vi "CSE Callback - Dialog Debugger.vi"(6 "Custom data":string, 7 "VC Handle":T2=-1, 8 "error in":errorcluster, 9 "Call Reason":T1=1 items=["Exec Start", "Action completed", "pause to breath", "reserved 1", "reserved 2", "custom"], 10 "Stm Index":i32, 11 "CSE RefNum":T3) -> (0 "error out":errorcluster, 1 "Run Mode":T4 items=["Execute", "Abort", "Run", "Step", "Step Over", "Step Out", "Run (LM)", "Step (LM)", "Step Over (LM)", "Step Out (LM)", "unsupported"], 2 "Stm Index out":i32, 3 "dup CSE RefNum":T3, 4 "Breakpoints":i32[](array[numeric]), 5 "VC Handle out":T2=-1)   [LabVIEW 2021]
doc: "::: CalcExpress Toolkit :::\nCopyright (c) 2000-2026 Konstantin Shifershteyn. All rights reserved."
uses:
  vi.lib/addons/CalcExpress/cse.llb/CSE Instance RefNum.ctl
  vi.lib/addons/CalcExpress/cetypes.llb/VarMan Variable Context Handle.ctl
  vi.lib/addons/CalcExpress/cse.llb/CSE Type - Run Mode.ctl
  vi.lib/addons/CalcExpress/cse.llb/CSE Type - Callback Call Reason.ctl
  <vilib>/Utility/miscctls.llb/LVRowAndColumnTypeDef.ctl
panel:
  in  "Quick exit":bool
  in  "Exit":bool caption="EXIT"
  in  "Breakpoint":bool caption="Set Breakpoint"
  in  "Stop":bool caption="Stop Debugging"
  in  "Pause":bool
  in  "Stepping mode":bool=TRUE
  in  "Restart":bool caption="Restart Script"
  in  "GoToCursor":bool caption="Go to Cursor"
  in  "StepOut":bool caption="Step Out"
  in  "StepOver":bool caption="Step Over"
  in  "Step":bool caption="Single Step"
  in  "Run":bool caption="Run Script"
  in  "Script List":i32(listbox) caption="Script"
  out "msg":string caption="Status message"
  in  "Var List":i32(listbox) caption="Variable List (inspect variables by double-click)"
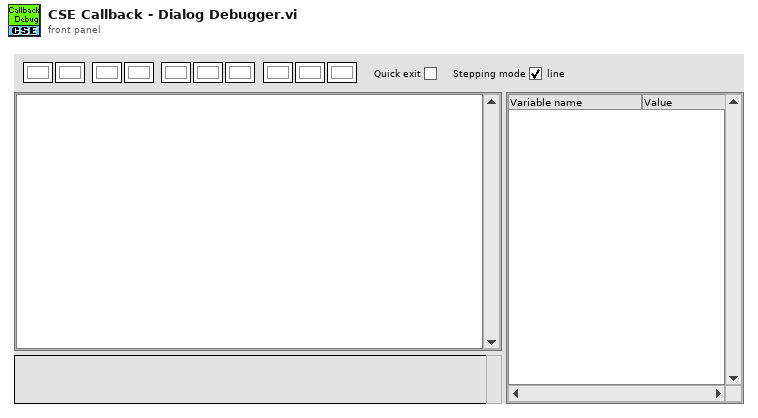
[diagram p1: front panel]
types:
  T1 = typedef "CSE Type - Callback Call Reason.ctl" = u32
  T2 = typedef "VarMan Variable Context Handle.ctl" = i32
  T3 = typedef "CSE Instance RefNum.ctl" = refnum<k1>
  T4 = typedef "CSE Type - Run Mode.ctl" = u32
  T5 = typedef "LVRowAndColumnTypeDef.ctl" = cluster{"Row":i32, "Column":i32}
  T6 = enum32{"nop", "save info", "restore info", "remove info"}
  T7 = cluster{"Selection Start":u32, "Selection End":u32}
  T8 = cluster{"level":i32, "Caller CSE RefNum":T3, "Callee CSE RefNum":T3}
  T9 = typedef "CalcExpress Instance RefNum.ctl" = refnum<k1>
  T10 = cluster{"CE InstanceRef":T9, "post action":enum32{"jump", "jump if true", "jump if false", "stop"}, "jump index":i32, "stmType":i32, "nesting level":i32, "stmOffset":i32, "stmLength":i32, "stmLine ":i32, "expOffset":i32, "expLength":i32, "expLine":i32, "parent index":i32}
  T11 = typedef "LVRowAndColumnUnsignedTypeDef.ctl" = cluster{"Row":u32, "Column":u32}
  T12 = typedef "VarMan Variable Info Cluster.ctl" = cluster{"name":string, "alias":string, "type":u32, "history":bool}
  T13 = enum8{"Enabled", "Disabled", "Disabled and Grayed Out"}
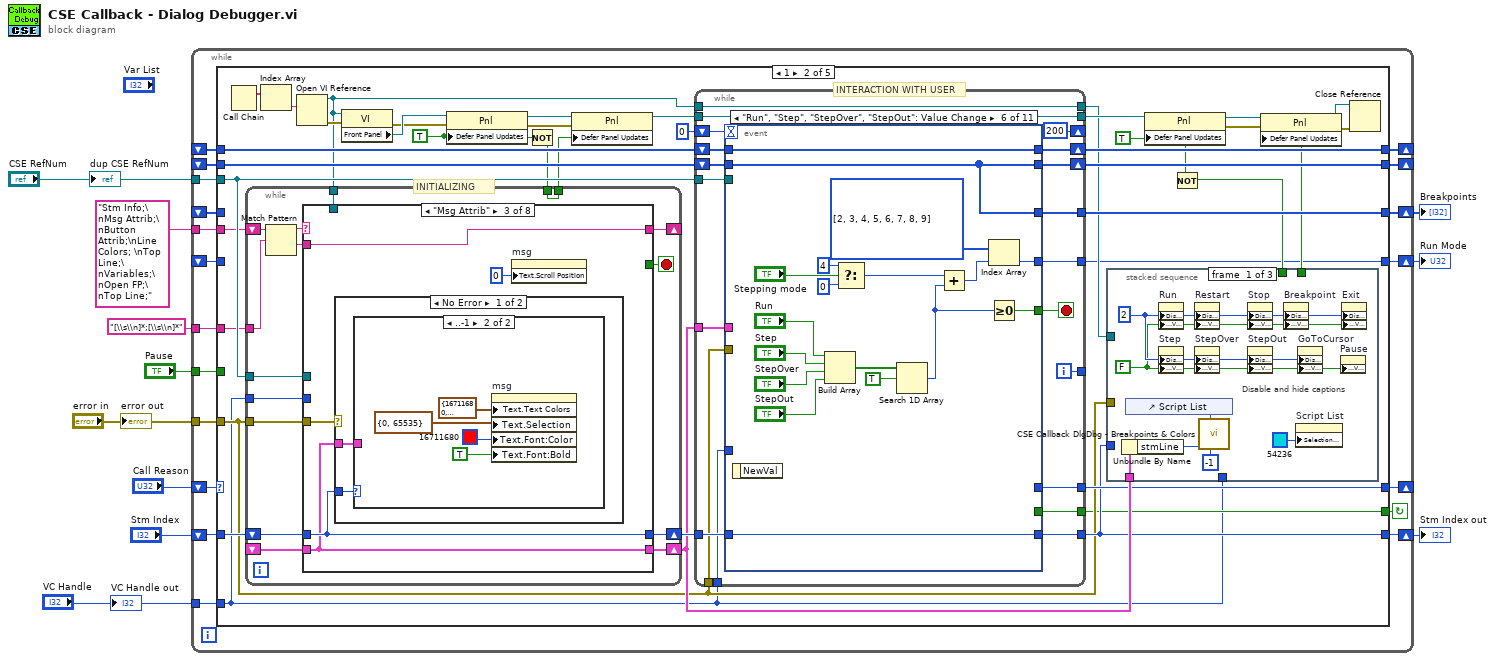
[diagram p0: block diagram]
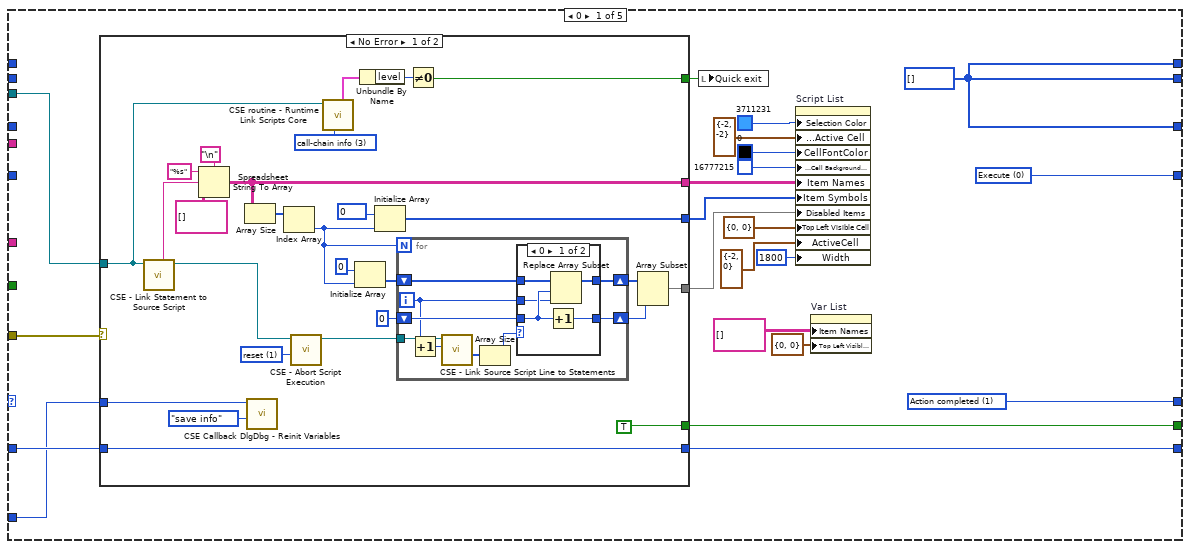
[diagram p2: hidden frame]
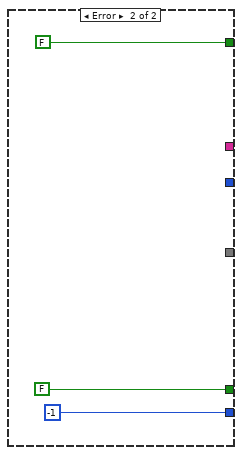
[diagram p4: hidden frame]
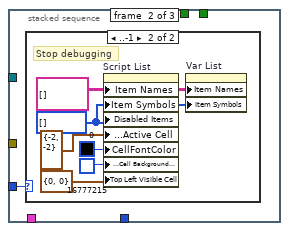
[diagram p5: hidden frame]
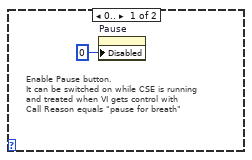
[diagram p6: hidden frame]
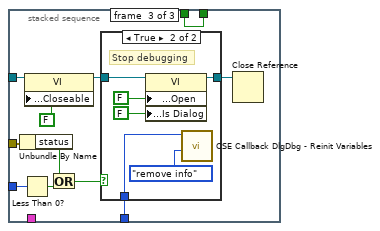
[diagram p7: hidden frame]
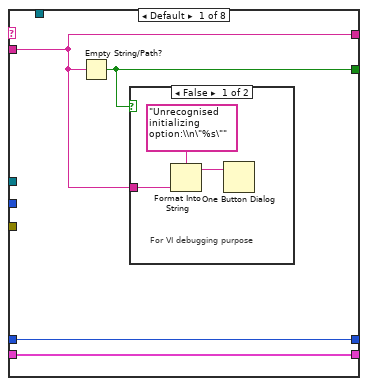
[diagram p9: hidden frame]
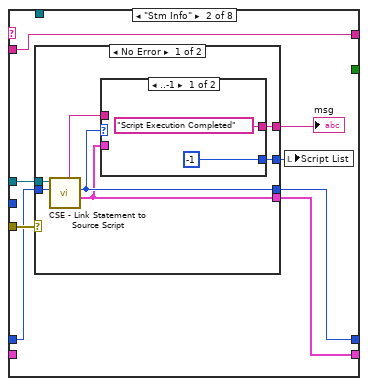
[diagram p11: hidden frame]
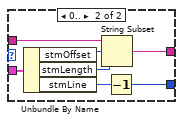
[diagram p12: hidden frame]
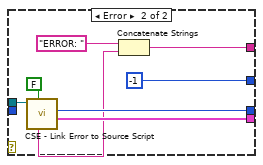
[diagram p13: hidden frame]
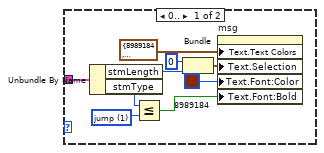
[diagram p14: hidden frame]
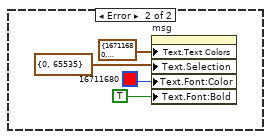
[diagram p15: hidden frame]
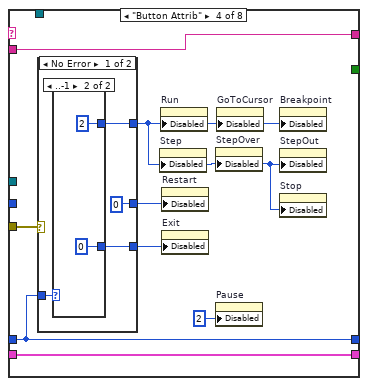
[diagram p16: hidden frame]
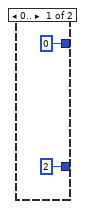
[diagram p17: hidden frame]
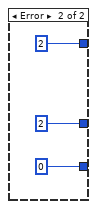
[diagram p18: hidden frame]
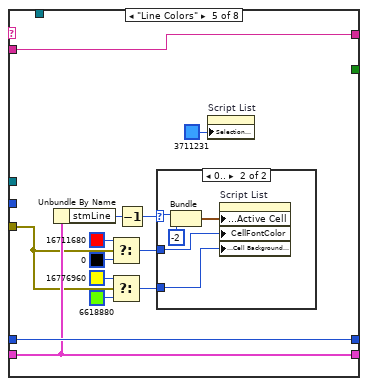
[diagram p19: hidden frame]
diagram:
  n1 = while {
    shift-right: [w29] -> _
    shift-left: "Call Reason" -> [w30]
    tunnel: "error in" -> [w27]
    tunnel: "CSE RefNum" -> [w26]
    shift-right: [w25] -> _
    shift-left: _ -> [w24]
    tunnel: "[\\s\\n]*;[\\s\\n]*" ("regular expression") -> [w23]
    tunnel: "Stm Info;\nMsg Attrib;\nButton Attrib;\nLine Colors; \nTop Line;\nVariables;\nOpen FP;\nTop Line;" -> [w22]
    shift-right: [w20] -> w5
    shift-left: "Stm Index" -> [w21]
    tunnel: "VC Handle" -> [w19]
    shift-right: [w18] -> _
    shift-left: _ -> [w17]
    tunnel: "Pause" -> [w16]
    shift-right: [w15] -> w2
    shift-left: _ -> [w13]
    shift-right: [w14] -> w1
    shift-left: _ -> [w12]
    stop <- w28 continue-if-true
    n2 = case shown="1" w30 {
      tunnel: [w36 w126 w549 _ _] -> w29
      tunnel: [w49 w103 w552 _ _] -> w28
      tunnel: [w37 w136 w550 w557 w564] -> w14
      tunnel: [w35 w102 w551 w556 w563] -> w15
      tunnel: w27 -> [w51 w104 _ _ _]
      tunnel: w26 -> [w52 w133 _ _ _]
      tunnel: [w37 w135 w555 w560 w567] -> w25
      tunnel: w24 -> [_ w134 w555 w560 w567]
      tunnel: w23 -> [_ w132 _ _ _]
      tunnel: w22 -> [_ w131 _ _ _]
      tunnel: w21 -> [w50 w130 w554 w559 w566]
      tunnel: [w48 w125 w554 w559 w566] -> w20
      tunnel: w19 -> [w34 w100 _ _ _]
      tunnel: [w37 w128 w553 w558 w565] -> w18
      tunnel: w17 -> [_ w127 w553 w558 w565]
      tunnel: w16 -> [_ _ w552 _ _]
      tunnel: w13 -> [_ _ w551 w556 w563]
      tunnel: w12 -> [_ _ w550 w557 w564]
      frame 0 {
        w37 = i32[] [] ("BreakPoints")
        w35 = T4 0 items=["Execute", "Abort", "Run", "Step", "Step Over", "Step Out", "Run (LM)", "Step (LM)", "Step Over (LM)", "Step Out (LM)", "unsupported"] ("Run Mode")
        w36 = T1 1 items=["Exec Start", "Action completed", "pause to breath", "reserved 1", "reserved 2", "custom"] ("Call Reason")
        n3 = case shown="No Error" w51 {
          tunnel: w52 -> [w55 _]
          tunnel: w50 -> [w67 _]
          tunnel: [w67 -1 ("Stm Index")] -> w48
          tunnel: [TRUE FALSE] -> w49
          tunnel: [w65 _] -> w41
          tunnel: [w64 _] -> w40
          tunnel: [w63 _] -> w39
          tunnel: w34 -> [w60 _]
          tunnel: [w53 FALSE] -> w33
          frame No Error {
            w58 = 3 items=["save vi path", "link to caller", "delink of caller", "call-chain info"] ("action")
            w62 = 1 items=["trigger", "reset", "check", "flip"] ("action")
            n4 = call "CSE - Link Statement to Source Script.vi"("CSE RefNum"=w55) -> ("dup CSE RefNum"=w61:T3, "script"=w68:string)  [unwired: 5 in, 4 out]
            n5 = Spreadsheet String To Array(delimiter (Tab)="\n", format string="%s", spreadsheet string=w68, array type (2D Dbl)=string[][] []) -> (array=w65:string[][])
            n6 = Array Size(array=w65) -> (size(s)=w75:i32[])
            n7 = call "CSE Callback DlgDbg - Reinit Variables.vi"("action"=T6."save info", "VC Handle"=w60) -> ()  [unwired: 8 in, 2 out]
            n8 = Index Array(array=w75) -> (element=w69:i32)  [unwired: 1 in]
            n9 = call "CSE - Abort Script Execution.vi"("action"=w62, "CSE RefNum"=w61) -> ("dup CSE RefNum"=w56:T3)  [unwired: 5 in, 2 out]
            n10 = call "CSE routine - Runtime Link Scripts Core.vi"("action"=w58, "CSE RefNum"=w55) -> ("call-chain info"=w57:T8)  [unwired: 4 in, 5 out]
            n11 = Initialize Array(0, w69) -> (w73:i32[])
            n12 = Unbundle By Name(w57) -> ("level"=w54:i32)
            n13 = Initialize Array(0, w69) -> (w64:i32[])
            n14 = for {
              N: w69 -> [_]
              shift-right: [w81] -> w71
              shift-left: w73 -> [w82]
              shift-right: [w83] -> w70
              shift-left: 0 -> [w84]
              tunnel: w56 -> [w88]
              i -> [w80]
              n15 = Increment(x=w80) -> (x+1=w87:i32)
              n16 = call "CSE - Link Source Script Line to Statements.vi"("Line number (1)"=w87, "CSE RefNum"=w88) -> ("Stm Indexes"=w86:i32[])  [unwired: 6 in, 3 out]
              n17 = Array Size(array=w86) -> (size(s)=w85:i32)
              n18 = case shown="0" w85 {
                tunnel: w84 -> [w90 w95]
                tunnel: [w91 w95] -> w83
                tunnel: w82 -> [w93 w94]
                tunnel: [w92 w94] -> w81
                tunnel: w80 -> [w89 _]
                frame 0 {
                  n19 = Increment(x=w90) -> (x+1=w91:i32)
                  n20 = Replace Array Subset(array=w93, new element=w89, index=w90) -> (w92:i32[])
                }
                frame 1, Default {
                }
              }
            }
            n21 = Not Equal To 0?(x=w54) -> (x != 0?=w53:bool)
            n22 = Array Subset(array=w71, length=w70) -> (w63:i32[])  [unwired: 1 in]
          }
          frame Error {
          }
        }
        n23 = local write "Quick exit"(w33) -> ()
        n24 = property on="Script List" class="MCListbox (strict)"("Selection Color"=u32 3711231, "Active Cell:Active Cell"=cluster{i32, i32} {-2, -2} ("Active Cell"), "CellFontColor"=u32 0, "Active Cell:Cell Background Color"=u32 16777215, "Item Names"=w41, "Item Symbols"=w40, "Disabled Items"=w39, "Top Left Visible Cell"=cluster{u32, u32} {0, 0}, "ActiveCell"=T5 {"Row"=-2, "Column"=0} ("Active Cell:Active Cell"), "Width"=u32 1800 ("Active Cell:Cell Size:Width")) -> ()  [unwired: 2 in, 2 out]
        n25 = property on="Var List" class="MCListbox (strict)"("Item Names"=string[][] [], "Top Left Visible Cell"=cluster{u32, u32} {0, 0}) -> ()  [unwired: 2 in, 2 out]
      }
      frame 1 {
        w111 = TRUE ("Defer Panel Updates")
        w118 = TRUE ("Defer Panel Updates")
        # "INTERACTION WITH USER"
        # "INITIALIZING"
        n26 = Call Chain() -> (call chain=w124:string[])
        n27 = Index Array(array=w124) -> (element=w99:string)  [unwired: 1 in]
        n28 = Open VI Reference(vi path=w99) -> (vi reference=w106:refnum<vi>, error out=w123:errorcluster)  [unwired: 5 in]
        n29 = property class="VI"(reference=w106, error in=w123) -> (error out=w121:errorcluster, "Front Panel"=w122:refnum<vi>)  [unwired: 1 out]
        n30 = property class="Pnl"(reference=w122, error in=w121, "Defer Panel Updates"=w118) -> (reference out=w120:refnum<vi>, error out=w119:errorcluster)
        n31 = Not(x=w118) -> (.not. x?=w117:bool)
        n32 = while {
          shift-right: [w185] -> w137
          shift-left: w130 -> [w183]
          shift-right: [w184] -> w129
          shift-left: _ -> [w182]
          tunnel: w104 -> [w181]
          tunnel: w133 -> [w180]
          shift-right: [w176] -> _
          shift-left: w131 -> [w178]
          tunnel: w132 -> [w175]
          tunnel: w100 -> [w173]
          tunnel: w117 -> [w172]
          tunnel: [w172] -> w116
          tunnel: w106 -> [w171]
          stop <- w174 stop-if-true
          n33 = Match Pattern(string=w178, regular expression=w175) -> (before substring=w179:string, after substring=w177:string)  [unwired: 1 in, 2 out]
          n34 = case shown="\"Msg Attrib\"" w179 {
            tunnel: [w189 w197 w227 w253 w280 w292 w324 w363] -> w185
            tunnel: [w188 w195 w226 w255 w279 w290 w323 w368] -> w184
            tunnel: w183 -> [w189 w196 w227 w253 w280 w292 w324 w363]
            tunnel: w182 -> [w188 _ w226 w255 w279 w290 w323 w368]
            tunnel: w181 -> [_ w200 w228 w254 w276 _ _ w366]
            tunnel: w180 -> [_ w199 _ _ _ _ _ _]
            tunnel: w177 -> [w186 w194 w229 w256 w277 w289 w325 w367]
            tunnel: [w186 w194 w229 w256 w277 w289 w325 w367] -> w176
            tunnel: [w187 _ _ _ _ _ _ _] -> w174
            tunnel: w173 -> [_ _ _ _ _ _ w322 _]
            tunnel: w171 -> [_ _ _ _ _ _ _ w361]
            frame Default {
              n35 = Empty String/Path?(string/path=w186) -> (empty?=w187:bool)
              n36 = case shown="False" w187 {
                tunnel: w186 -> [w191 _]
                frame False {
                  # "For VI debugging purpose"
                  n37 = Format Into String(format string="Unrecognised initializing option:\\n\"%s\"", w191) -> (resulting string=w190:string)  [unwired: 2 in, 1 out]
                  n38 = One Button Dialog(message=w190) -> ()  [unwired: 1 in, 1 out]
                }
                frame True {
                }
              }
            }
            frame "Stm Info" {
              n39 = case shown="No Error" w200 {
                tunnel: w199 -> [w207 w224]
                tunnel: [w202 w223] -> w195
                tunnel: w196 -> [w206 _]
                tunnel: [w204 w222] -> w197
                tunnel: [w203 w220] -> w198
                tunnel: [w201 -1 ("script-list")] -> w193
                frame No Error {
                  n40 = call "CSE - Link Statement to Source Script.vi"("Stm Index"=w206, "CSE RefNum"=w207) -> ("statement info"=w202:T10, "dup Stm Index"=w204:i32, "script"=w205:string)  [unwired: 4 in, 3 out]
                  n41 = case shown="..-1" w204 {
                    tunnel: w205 -> [_ w214]
                    tunnel: ["Script Execution Completed" ("script") w213] -> w203
                    tunnel: w202 -> [_ w212]
                    tunnel: [-1 ("stmLine") w210] -> w201
                    frame ..-1 {
                    }
                    frame 0.. {
                      n42 = Unbundle By Name(w212) -> ("stmOffset"=w216:i32, "stmLength"=w215:i32, "stmLine"=w211:i32)
                      n43 = String Subset(string=w214, offset (0)=w216, length (rest)=w215) -> (substring=w213:string)
                      n44 = Decrement(x=w211) -> (x-1=w210:i32)
                    }
                  }
                }
                frame Error {
                  n45 = call "CSE - Link Error to Source Script.vi"("get script source (T)"=FALSE, "CSE RefNum"=w224) -> ("statement info"=w223:T10, "Stm Index"=w222:i32, "Error Message"=w219:string)  [unwired: 3 in, 4 out]
                  n46 = Concatenate Strings("ERROR: " ("string"), w219) -> (w220:string)
                }
              }
              "msg" <- w198
              n47 = local write "Script List"(w193) -> ()
            }
            frame "Msg Attrib" {
              n48 = case shown="No Error" w228 {
                tunnel: w227 -> [w231 _]
                tunnel: w226 -> [w230 _]
                frame No Error {
                  n49 = case shown="..-1" w231 {
                    tunnel: w230 -> [w233 _]
                    frame 0.. {
                      w237 = 1 items=["expression", "jump", "source ref", "jump stub", "source stub"] ("stmType")
                      n50 = Unbundle By Name(w233) -> ("stmLength"=w235:i32, "stmType"=w238:i32)
                      n51 = Less Or Equal?(x=w238, y=w237) -> (x <= y?=w234:bool)
                      n52 = Bundle(0, "stmLength"=w235) -> (w240:cluster{i32, "stmLength":i32})  [unwired: 1 in]
                      n53 = property on="msg" class="Str"("Text.Text Colors"=cluster{u32, u32} {8989184, 16777215}, "Text.Selection"=w240, "Text.Font:Color"=u32 8989184, "Text.Font:Bold"=w234) -> ()  [unwired: 2 in, 2 out]
                    }
                    frame ..-1 {
                      n54 = property on="msg" class="Str"("Text.Text Colors"=cluster{u32, u32} {16711680, 16515000}, "Text.Selection"=T7 {"Selection Start"=0, "Selection End"=65535}, "Text.Font:Color"=u32 16711680, "Text.Font:Bold"=TRUE) -> ()  [unwired: 2 in, 2 out]
                    }
                  }
                }
                frame Error {
                  n55 = property on="msg" class="Str"("Text.Text Colors"=cluster{u32, u32} {16711680, 16776960}, "Text.Selection"=T7 {"Selection Start"=0, "Selection End"=65535}, "Text.Font:Color"=u32 16711680, "Text.Font:Bold"=TRUE) -> ()  [unwired: 2 in, 2 out]
                }
              }
              n56 = property on="msg" class="Str"("Text.Scroll Position"=u32 0) -> ()  [unwired: 2 in, 2 out]
            }
            frame "Button Attrib" {
              n57 = case shown="No Error" w254 {
                tunnel: w253 -> [w260 _]
                tunnel: [w259 u8 2 ("Disabled")] -> w249
                tunnel: [u8 0 ("Disabled") u8 2 ("Disabled")] -> w252
                tunnel: [w257 u8 0 ("Disabled")] -> w250
                frame No Error {
                  n58 = case shown="..-1" w260 {
                    tunnel: [u8 0 ("Disabled") u8 2 ("Disabled")] -> w259
                    tunnel: [u8 2 ("Disabled") u8 0 ("Disabled")] -> w257
                    frame 0.. {
                    }
                    frame ..-1 {
                    }
                  }
                }
                frame Error {
                }
              }
              n59 = property on="Step" class="Bool"("Disabled"=w249) -> ()  [unwired: 2 in, 2 out]
              n60 = property on="Run" class="Bool"("Disabled"=w249) -> ()  [unwired: 2 in, 2 out]
              n61 = property on="Restart" class="Bool"("Disabled"=w252) -> ()  [unwired: 2 in, 2 out]
              n62 = property on="Exit" class="Bool"("Disabled"=w250) -> ()  [unwired: 2 in, 2 out]
              n63 = property on="StepOver" class="Bool"("Disabled"=w249) -> ()  [unwired: 2 in, 2 out]
              n64 = property on="Pause" class="Bool"("Disabled"=u8 2) -> ()  [unwired: 2 in, 2 out]
              n65 = property on="GoToCursor" class="Bool"("Disabled"=w249) -> ()  [unwired: 2 in, 2 out]
              n66 = property on="Breakpoint" class="Bool"("Disabled"=w249) -> ()  [unwired: 2 in, 2 out]
              n67 = property on="StepOut" class="Bool"("Disabled"=w249) -> ()  [unwired: 2 in, 2 out]
              n68 = property on="Stop" class="Bool"("Disabled"=w249) -> ()  [unwired: 2 in, 2 out]
            }
            frame "Line Colors" {
              n69 = Unbundle By Name(w279) -> ("stmLine"=w278:i32)
              n70 = Select(t=u32 16711680, s=w276, f=u32 0) -> (s? t:f=w271:u32)
              n71 = Select(t=u32 16776960, s=w276, f=u32 6618880) -> (s? t:f=w270:u32)
              n72 = Decrement(x=w278) -> (x-1=w269:i32)
              n73 = case shown="0.." w269 {
                selector: w269 -> [_ w281]
                tunnel: w271 -> [_ w283]
                tunnel: w270 -> [_ w282]
                frame ..-1 {
                }
                frame 0.. {
                  n74 = Bundle(w281, -2) -> (w284:cluster{i32, i32})  [unwired: 1 in]
                  n75 = property on="Script List" class="MCListbox (strict)"("Active Cell:Active Cell"=w284, "CellFontColor"=w283, "Active Cell:Cell Background Color"=w282) -> ()  [unwired: 2 in, 2 out]
                }
              }
              n76 = property on="Script List" class="MCListbox (strict)"("Selection Color"=u32 3711231) -> ()  [unwired: 2 in, 2 out]
            }
            frame "Top Line" {
              n77 = Unbundle By Name(w290) -> ("stmLine"=w291:i32)
              n78 = property on="Script List" class="MCListbox (strict)"() -> ("Top Left Visible Cell"=w287:T11, "Number of Rows"=w286:u32)  [unwired: 2 in, 2 out]
              n79 = Decrement(x=w291) -> (x-1=w288:i32)
              n80 = case shown="0.." w288 {
                selector: w288 -> [w300 _]
                tunnel: w287 -> [w299 _]
                tunnel: w286 -> [w297 _]
                frame 0.. {
                  n81 = Decrement(x=w297) -> (x-1=w293:u32)
                  n82 = Unbundle(w299) -> ("Row"=w301:u32)  [unwired: 1 out]
                  n83 = To Unsigned Long Integer(number=w300) -> (unsigned 32bit integer=w296:u32)
                  n84 = Add(x=w301, y=w293) -> (x+y=w302:u32)
                  n85 = Less?(x=w296, y=w301) -> (x < y?=w295:bool)
                  n86 = Greater Or Equal?(x=w296, y=w302) -> (x >= y?=w294:bool)
                  n87 = Or(x=w295, y=w294) -> (x .or. y?=w298:bool)
                  n88 = case shown="True" w298 {
                    tunnel: w293 -> [_ w308]
                    tunnel: w296 -> [_ w307]
                    tunnel: w294 -> [_ w306]
                    frame False {
                    }
                    frame True {
                      n89 = case shown="True" w306 {
                        tunnel: w307 -> [w311 w316]
                        tunnel: [w309 w314] -> w303
                        tunnel: w308 -> [_ w315]
                        frame False {
                          n90 = Decrement(x=w311) -> (x-1=w310:u32)
                          n91 = Max & Min(x=w310, y=w311) -> (min(x,y)=w309:u32)  [unwired: 1 out]
                        }
                        frame True {
                          n92 = Subtract(x=w316, y=w315) -> (x-y=w313:u32)
                          n93 = Add(x=u32 1 ("y"), y=w313) -> (x+y=w314:u32)
                        }
                      }
                      n94 = Bundle(w303, u32 0) -> (w304:cluster{u32, u32})  [unwired: 1 in]
                      n95 = property on="Script List" class="MCListbox (strict)"("Top Left Visible Cell"=w304) -> ()  [unwired: 2 in, 2 out]
                    }
                  }
                }
                frame ..-1 {
                }
              }
            }
            frame "Variables" {
              n96 = call "VM - List of Variables.vi"("sort"=enum16{"don't sort", "name", "alias", "type"}."name", "VC Handle"=w322) -> ("variables info"=w320:T12[], "dup VC Handle"=w319:T2)  [unwired: 5 in, 1 out]
              n97 = for {
                tunnel: w320 -> [w332] mode=indexing
                tunnel: w319 -> [w331]
                tunnel: [w329] -> w318 mode=indexing
                tunnel: [w328] -> w317 mode=indexing
                n98 = Unbundle By Name(w332) -> ("name"=w330:string, "type"=w327:u32)
                n99 = case shown="252" w327 {
                  tunnel: w330 -> [w335 w340 w345 _ _ w355 _]
                  tunnel: w331 -> [w334 w339 w344 _ _ w352 _]
                  tunnel: [w333 w337 w343 "[..]" "[[..]]" w354 "..."] -> w326
                  frame 0 {
                    n100 = call "VM - Strings.vi"("VC Handle"=w334, "name_spec"=w335) -> ("value out"=w333:string)  [unwired: 4 in, 5 out]
                  }
                  frame 1 {
                    n101 = call "VM - DBL Scalar.vi"("VC Handle"=w339, "name_spec"=w340) -> ("value out"=w338:dbl)  [unwired: 4 in, 5 out]
                    n102 = Format Value(format string="%.;%#_g", value (0)=w338) -> (output string=w337:string)  [unwired: 1 in]
                  }
                  frame 5 {
                    n103 = call "VM - CDB Scalar.vi"("VC Handle"=w344, "name_spec"=w345) -> ("value out"=w342:cdb)  [unwired: 4 in, 5 out]
                    n104 = Format Value(format string="%.;%#_g", value (0)=w342) -> (output string=w343:string)  [unwired: 1 in]
                  }
                  frame 3, 6, 8 {
                  }
                  frame 4, 7, 9 {
                  }
                  frame 252 {
                    n105 = call "VM - Arbitrary Data.vi"("var type"=u32 252, "VC Handle"=w352, "name_spec"=w355) -> ("flattened value out"=w351:string)  [unwired: 3 in, 5 out]
                    n106 = call "[ce] Index Range from Flattened String.vi"("Flattened string"=w351) -> ("Index Range"=w350:cluster{"Initial index":i32, "Final index":i32})  [unwired: 10 in]
                    n107 = Unbundle(w350) -> ("Initial index"=w349:i32, "Final index"=w348:i32)
                    n108 = Format Into String(format string="{%d:%d}", w349, w348) -> (resulting string=w354:string)  [unwired: 2 in, 1 out]
                  }
                  frame Default {
                  }
                }
                n109 = call "CSE ISP - VM Datatype to List Symbol.vi"("VarMan Datatype Code"=w327) -> ("List/Tree Symbol"=w328:i32)  [unwired: 10 in]
                n110 = Build Array(w330, w326) -> (w329:string[])
              }
              n111 = property on="Var List" class="MCListbox (strict)"("Item Names"=w318, "ItemSyms"=w317) -> ()  [unwired: 2 in, 2 out]
            }
            frame "Open FP" {
              n112 = Unbundle By Name(w366) -> ("status"=w365:bool)
              n113 = Less Than 0?(x=w363) -> (x < 0?=w364:bool)
              n114 = Or(x=w365, y=w364) -> (x .or. y?=w362:bool)
              n115 = property class="VI"(reference=w361, "Front Panel Window:Is Frontmost"=TRUE, "Front Panel Window:Closeable"=TRUE, "Front Panel Window:Is Dialog"=w362) -> (reference out=w359:refnum<vi>)  [unwired: 1 in, 1 out]
              n116 = invoke class="VI" method="FP.Open"(reference=w359, "Activate"=TRUE ("Activate?")) -> ()  [unwired: 3 in, 5 out]
            }
          }
        }
        n117 = property class="Pnl"(reference=w120, error in=w119, "Defer Panel Updates"=w116) -> (reference out=w113:refnum<vi>)  [unwired: 1 out]
        n118 = while {
          tunnel: [w388] -> w102
          tunnel: [w387] -> w136
          tunnel: w137 -> [w383]
          tunnel: w129 -> [w376]
          shift-right: [w385] -> w135
          shift-left: w134 -> [w386]
          tunnel: w133 -> [w384]
          tunnel: [w382] -> w125
          tunnel: [w381] -> w103
          tunnel: w100 -> [w380]
          shift-right: [w378] -> w128
          shift-left: w127 -> [w379]
          tunnel: [w377] -> w126
          tunnel: w113 -> [w375]
          tunnel: [w375] -> w112
          tunnel: w106 -> [w374]
          tunnel: [w374] -> w105
          tunnel: w104 -> [w373]
          shift-right: [200] -> _
          shift-left: 0 -> [w372]
          tunnel: [w371] -> _
          i -> [w371]
          stop <- w389 stop-if-true
          n119 = event shown="[5] \"Run\", \"Step\", \"StepOver\", \"StepOut\": Value Change" {
            selector: _ -> [_ _ _ _ _ _ _ _ _ _ _]
            dyn-events: _ -> [_ _ _ _ _ _ _ _ _ _ _]
            timeout: w372 -> [_ _ _ _ _ _ _ _ _ _ _]
            tunnel: [w392 w409 TRUE ("Discard?") TRUE ("Discard?") TRUE w456 w477 _ _ _ _] -> w389
            tunnel: [w405 w414 w424 w429 _ w446 w464 _ _ _ _] -> w388
            tunnel: [_ _ _ _ _ w454 w476 _ _ _ _] -> w387
            tunnel: w386 -> [w390 w417 w426 w431 w441 w454 w473 w488 w498 w515 w540]
            tunnel: [w390 w417 w426 w431 w441 w454 w473 w488 w495 w513 w540] -> w385
            tunnel: w384 -> [w407 w410 w423 _ _ _ w474 _ w492 w512 _]
            tunnel: w383 -> [w395 _ _ _ _ w463 w469 w490 w493 w519 w542]
            tunnel: [w395 -1 ("Stm Index") -1 ("Stm Index") -1 ("Stm Index") 0 ("Stm Index") w463 w469 w490 w493 w519 w542] -> w382
            tunnel: [_ _ _ _ TRUE _ _ _ _ _ _] -> w381
            tunnel: w380 -> [_ _ _ _ w437 _ _ _ _ _ w543]
            tunnel: w379 -> [w391 w415 w425 w430 w434 w455 w468 w489 w497 w516 w541]
            tunnel: [w391 w415 w425 w430 w434 w455 w468 w489 w496 w514 w541] -> w378
            tunnel: [_ _ _ _ w433 _ _ _ _ _ _] -> w377
            tunnel: w376 -> [_ _ _ _ _ _ _ _ w494 w518 _]
            tunnel: w373 -> [w403 _ _ _ _ _ _ _ _ _ _]
            event Timeout {
              w398 = 7104  # Abort
              w404 = 2 items=["trigger", "reset", "check", "flip"] ("action")
              w405 = T4 1 items=["Execute", "Abort", "Run", "Step", "Step Over", "Step Out", "Run (LM)", "Step (LM)", "Step Over (LM)", "Step Out (LM)", "unsupported"] ("Run Mode")
              n120 = event-data() -> ()  [unwired: 1 in, 1 out]
              n121 = Unbundle By Name(w403) -> ("status"=w400:bool, "code"=w402:i32)
              n122 = Less Than 0?(x=w395) -> (x < 0?=w396:bool)
              n123 = call "CSE - Abort Script Execution.vi"("action"=w404, "CSE RefNum"=w407) -> ("triggered"=w406:bool)  [unwired: 5 in, 2 out]
              n124 = Equal?(x=w402, y=w398) -> (x = y?=w401:bool)
              n125 = And(x="Quick exit", y=w396) -> (x .and. y?=w393:bool)
              n126 = And(x=w400, y=w401) -> (x .and. y?=w399:bool)
              n127 = Or(x=w406, y=w399) -> (x .or. y?=w394:bool)
              n128 = Or(x=w394, y=w393) -> (x .or. y?=w392:bool)
            }
            event Panel Close? {
              w414 = T4 1 items=["Execute", "Abort", "Run", "Step", "Step Over", "Step Out", "Run (LM)", "Step (LM)", "Step Over (LM)", "Step Out (LM)", "unsupported"] ("Run Mode")
              # "This is made in order to prevent \n\"Save changes\" request when FP is closed"
              n129 = event-data() -> ()  [unwired: 1 in, 1 out]
              n130 = property on="Run" class="Bool"() -> ("DisabledEnum"=w412:T13)  [unwired: 2 in, 2 out]
              n131 = case shown="\"Enabled\"" w412 {
                tunnel: [w419 TRUE ("T button?")] -> w409
                tunnel: "This operation will terminate the debugging session.\nAre you sure?" -> [w420 _]
                tunnel: [w419 _] -> w408
                frame "Enabled" {
                  n132 = Two Button Dialog(message=w420) -> (T button?=w419:bool)  [unwired: 2 in]
                }
                frame Default {
                }
              }
              n133 = case shown="True" w408 {
                tunnel: w410 -> [_ w418]
                frame False {
                }
                frame True {
                  n134 = call "CSE - Abort Script Execution.vi"("CSE RefNum"=w418) -> ()  [unwired: 6 in, 3 out]
                }
              }
              n135 = event-data("Discard?"=TRUE) -> ()  [unwired: 1 in, 1 out]
            }
            event "Stop": Value Change {
              w424 = T4 1 items=["Execute", "Abort", "Run", "Step", "Step Over", "Step Out", "Run (LM)", "Step (LM)", "Step Over (LM)", "Step Out (LM)", "unsupported"] ("Run Mode")
              n136 = event-data() -> ()  [unwired: 1 in, 1 out]
              n137 = call "CSE - Abort Script Execution.vi"("CSE RefNum"=w423) -> ()  [unwired: 6 in, 3 out]
            }
            event "Exit": Value Change {
              w429 = T4 0 items=["Execute", "Abort", "Run", "Step", "Step Over", "Step Out", "Run (LM)", "Step (LM)", "Step Over (LM)", "Step Out (LM)", "unsupported"] ("Run Mode")
              n138 = event-data() -> ()  [unwired: 1 in, 1 out]
            }
            event "Restart": Value Change {
              w433 = T1 1 items=["Exec Start", "Action completed", "pause to breath", "reserved 1", "reserved 2", "custom"] ("Call Reason")
              n139 = event-data() -> ()  [unwired: 1 in, 1 out]
              n140 = Two Button Dialog(message="Restore original variables?", 1:"No" ("F button name (\"Cancel\")"), 2:"Yes" ("T button name (\"OK\")")) -> (T button?=w438:bool)
              n141 = case shown="True" w438 {
                tunnel: w437 -> [_ w445]
                frame False {
                }
                frame True {
                  n142 = call "CSE Callback DlgDbg - Reinit Variables.vi"("action"=T6."restore info", "VC Handle"=w445) -> ()  [unwired: 8 in, 2 out]
                }
              }
            }
            event "Run", "Step", "StepOver", "StepOut": Value Change {
              w447 = T4[] [2, 3, 4, 5, 6, 7, 8, 9] items=["Execute", "Abort", "Run", "Step", "Step Over", "Step Out", "Run (LM)", "Step (LM)", "Step Over (LM)", "Step Out (LM)", "unsupported"]
              n143 = event-data() -> ()  [unwired: 1 in, 1 out]
              n144 = Build Array("Run", "Step", "StepOver", "StepOut") -> (w458:bool[])
              n145 = Select(t=4, s="Stepping mode", f=0) -> (s? t:f=w450:i32)
              n146 = Search 1D Array(1D array=w458, element=TRUE) -> (index of element=w449:i32)  [unwired: 1 in]
              n147 = Add(x=w450, y=w449) -> (x+y=w448:i32)
              n148 = Index Array(array=w447, index=w448) -> (element=w446:T4)
              n149 = Greater Or Equal To 0?(x=w449) -> (x >= 0?=w456:bool)
            }
            event "GoToCursor": Value Change {
              w466 = T4 6 items=["Execute", "Abort", "Run", "Step", "Step Over", "Step Out", "Run (LM)", "Step (LM)", "Step Over (LM)", "Step Out (LM)", "unsupported"] ("Run Mode")
              w465 = T4 2 items=["Execute", "Abort", "Run", "Step", "Step Over", "Step Out", "Run (LM)", "Step (LM)", "Step Over (LM)", "Step Out (LM)", "unsupported"] ("Run Mode")
              n150 = event-data() -> ()  [unwired: 1 in, 1 out]
              n151 = Increment(x="Script List") -> (x+1=w470:i32)
              n152 = call "CSE - Link Source Script Line to Statements.vi"("Line number (1)"=w470, "CSE RefNum"=w474) -> ("Stm Indexes"=w472:i32[])  [unwired: 6 in, 3 out]
              n153 = local read "Stepping mode"() -> (w467:bool)
              n154 = Array Size(array=w472) -> (size(s)=w471:i32)
              n155 = case shown="1, Default" w471 {
                tunnel: [_ TRUE ("Discard?")] -> w477
                tunnel: [w479 w482] -> w476
                tunnel: w473 -> [w479 w481]
                tunnel: w472 -> [_ w480]
                frame 0 {
                  n156 = One Button Dialog(message="No valid statement in this line") -> ()  [unwired: 1 in, 1 out]
                }
                frame 1, Default {
                  n157 = Build Array (concatenate)(w481, w480) -> (w482:i32[])
                }
              }
              n158 = Select(t=w466, s=w467, f=w465) -> (s? t:f=w464:T4)
            }
            event "Script List": Value Change {
              n159 = event-data() -> ("NewVal"=w487:i32)  [unwired: 1 in]
              n160 = Less Than 0?(x=w487) -> (x < 0?=w486:bool)
              n161 = Boolean To (0,1)(Boolean=w486) -> (0, 1=w485:i16)
              n162 = Add(x=w485, y=w485) -> (x+y=w484:i16)
              n163 = property on="Breakpoint" class="Bool"("Disabled"=w484) -> ()  [unwired: 2 in, 2 out]
              n164 = property on="GoToCursor" class="Bool"("Disabled"=w484) -> ()  [unwired: 2 in, 2 out]
            }
            event "Script List": Double Click {
              n165 = event-data() -> ("Row"=w491:i32)  [unwired: 1 in]
              n166 = case shown="0.." w491 {
                selector: w491 -> [w503 _]
                tunnel: w498 -> [w508 w510]
                tunnel: w497 -> [w507 w511]
                tunnel: w492 -> [w506 _]
                tunnel: [w505 w511] -> w496
                tunnel: [w504 w510] -> w495
                tunnel: w494 -> [w500 _]
                frame 0.. {
                  n167 = control-ref of="Script List"() -> (w502:refnum<vi>)
                  n168 = Increment(x=w503) -> (x+1=w509:i32)
                  n169 = Unbundle By Name(w500) -> ("stmLine"=w501:i32)
                  n170 = call "CSE Callback DlgDbg - Breakpoints & Colors.vi"("Treat breakpoint"=TRUE, "Current Stm Line"=w501, "MCListbox Refnum"=w502, "Line Number (1)"=w509, "Stm Idxs"=w508, "Line Nums"=w507, "CSE RefNum"=w506) -> ("Stm Idxs out"=w504:i32[], "Line Nums out"=w505:i32[])  [unwired: 2 in, 1 out]
                }
                frame ..-1 {
                }
              }
            }
            event "Breakpoint": Value Change {
              n171 = event-data() -> ()  [unwired: 1 in, 1 out]
              n172 = local read "Script List"() -> (w517:i32)
              n173 = case shown="0.." w517 {
                selector: w517 -> [w524 _]
                tunnel: w515 -> [w529 w531]
                tunnel: w516 -> [w528 w532]
                tunnel: w512 -> [w527 _]
                tunnel: [w526 w532] -> w514
                tunnel: [w525 w531] -> w513
                tunnel: w518 -> [w521 _]
                frame 0.. {
                  n174 = control-ref of="Script List"() -> (w523:refnum<vi>)
                  n175 = Increment(x=w524) -> (x+1=w530:i32)
                  n176 = Unbundle By Name(w521) -> ("stmLine"=w522:i32)
                  n177 = call "CSE Callback DlgDbg - Breakpoints & Colors.vi"("Treat breakpoint"=TRUE, "Current Stm Line"=w522, "MCListbox Refnum"=w523, "Line Number (1)"=w530, "Stm Idxs"=w529, "Line Nums"=w528, "CSE RefNum"=w527) -> ("Stm Idxs out"=w525:i32[], "Line Nums out"=w526:i32[])  [unwired: 2 in, 1 out]
                }
                frame ..-1 {
                }
              }
            }
            event "Var List": Double Click {
              n178 = event-data() -> ("Row"=w539:i32)  [unwired: 1 in]
              n179 = property on="Var List" class="MCListbox (strict)"() -> ("Item Names"=w536:string[][])  [unwired: 2 in, 2 out]
              n180 = Array Size(array=w536) -> (size(s)=w537:i32[])
              n181 = Index Array(array=w537) -> (element=w534:i32)  [unwired: 1 in]
              n182 = In Range and Coerce(upper limit=w534, x=w539, lower limit=0) -> (coerced(x)=w538:i32, In Range?=w535:bool)
              n183 = case shown="True" w535 {
                tunnel: w543 -> [_ w548]
                tunnel: w538 -> [_ w545]
                tunnel: w536 -> [_ w544]
                frame False {
                }
                frame True {
                  n184 = Index Array(array=w544, index (row)=w545, index (col)=0 ("disabled index (col)")) -> (element=w547:string)
                  n185 = call "Inspector Launcher [VarMan Spy].vi"("VC Handle"=w548, "Variable"=w547) -> ()  [unwired: 7 in, 1 out]
                }
              }
            }
          }
        }
        n186 = property class="Pnl"(reference=w112, "Defer Panel Updates"=w111) -> (reference out=w114:refnum<vi>, error out=w115:errorcluster)  [unwired: 1 in]
        n187 = Not(x=w111) -> (.not. x?=w108:bool)
        n188 = stacked-sequence {
          tunnel: w129 -> [w144 _ _]
          tunnel: w125 -> [_ w145 w162]
          tunnel: [_ _ w154] -> w109
          tunnel: w108 -> [_ _ w154]
          tunnel: w105 -> [_ _ w156]
          tunnel: w104 -> [_ _ w163]
          tunnel: w100 -> [_ _ w153]
          frame #0 {
            w138 = FALSE
            w139 = u8 2 ("Disabled")
            # "Disable and hide captions"
            n189 = Unbundle By Name(w144) -> ("stmLine"=w143:i32)
            n190 = control-ref of="Script List"() -> (w141:refnum<vi>)
            n191 = property on="Run" class="Bool"("Disabled"=w139, "Caption.Visible"=w138) -> ()  [unwired: 2 in, 2 out]
            n192 = property on="Step" class="Bool"("Disabled"=w139, "Caption.Visible"=w138) -> ()  [unwired: 2 in, 2 out]
            n193 = property on="Restart" class="Bool"("Disabled"=w139, "Caption.Visible"=w138) -> ()  [unwired: 2 in, 2 out]
            n194 = property on="StepOver" class="Bool"("Disabled"=w139, "Caption.Visible"=w138) -> ()  [unwired: 2 in, 2 out]
            n195 = call "CSE Callback DlgDbg - Breakpoints & Colors.vi"("Current Stm Line"=-1, "MCListbox Refnum"=w141, "Line Number (1)"=w143) -> ()  [unwired: 6 in, 3 out]
            n196 = property on="Stop" class="Bool"("Disabled"=w139, "Caption.Visible"=w138) -> ()  [unwired: 2 in, 2 out]
            n197 = property on="StepOut" class="Bool"("Disabled"=w139, "Caption.Visible"=w138) -> ()  [unwired: 2 in, 2 out]
            n198 = property on="Breakpoint" class="Bool"("Disabled"=w139, "Caption.Visible"=w138) -> ()  [unwired: 2 in, 2 out]
            n199 = property on="Script List" class="MCListbox (strict)"("Selection Color"=u32 54236) -> ()  [unwired: 2 in, 2 out]
            n200 = property on="GoToCursor" class="Bool"("Disabled"=w139, "Caption.Visible"=w138) -> ()  [unwired: 2 in, 2 out]
            n201 = property on="Pause" class="Bool"("Caption.Visible"=w138) -> ()  [unwired: 2 in, 2 out]
            n202 = property on="Exit" class="Bool"("Disabled"=w139, "Caption.Visible"=w138) -> ()  [unwired: 2 in, 2 out]
          }
          frame #1 {
            n203 = case shown="..-1" w145 {
              frame 0.. {
                # "Enable Pause button.\nIt can be switched on while CSE is running\nand treated when VI gets control with\nCall Reason equals \"pause for breath\""
                n204 = property on="Pause" class="Bool"("Disabled"=u8 0) -> ()  [unwired: 2 in, 2 out]
              }
              frame ..-1 {
                w151 = i32[] [] ("Item Symbols")
                w152 = string[][] [] ("Item Names")
                # "Stop debugging"
                n205 = property on="Script List" class="MCListbox (strict)"("Item Names"=w152, "Item Symbols"=w151, "Disabled Items"=w151, "Active Cell:Active Cell"=cluster{i32, i32} {-2, -2} ("Active Cell"), "CellFontColor"=u32 0, "Active Cell:Cell Background Color"=u32 16777215, "Top Left Visible Cell"=cluster{u32, u32} {0, 0}) -> ()  [unwired: 2 in, 2 out]
                n206 = property on="Var List" class="MCListbox (strict)"("Item Names"=w152, "Item Symbols"=w151) -> ()  [unwired: 2 in, 2 out]
              }
            }
          }
          frame #2 {
            n207 = Unbundle By Name(w163) -> ("status"=w160:bool)
            n208 = Less Than 0?(x=w162) -> (x < 0?=w161:bool)
            n209 = property class="VI"(reference=w156, "Front Panel Window:Closeable"=FALSE) -> (reference out=w157:refnum<vi>)  [unwired: 1 in, 1 out]
            n210 = Or(x=w160, y=w161) -> (x .or. y?=w159:bool)
            n211 = case shown="True" w159 {
              tunnel: w157 -> [w164 w168]
              tunnel: [w164 w167] -> w155
              tunnel: w153 -> [_ w166]
              frame False {
              }
              frame True {
                # "Stop debugging"
                n212 = property class="VI"(reference=w168, "Front Panel Window:Open"=FALSE, "Front Panel Window:Is Dialog"=FALSE) -> (reference out=w167:refnum<vi>)  [unwired: 1 in, 1 out]
                n213 = call "CSE Callback DlgDbg - Reinit Variables.vi"("action"=T6."remove info", "VC Handle"=w166) -> ()  [unwired: 8 in, 2 out]
              }
            }
            n214 = Close Reference(reference=w155) -> ()  [unwired: 1 in, 1 out]
          }
        }
        n215 = property class="Pnl"(reference=w114, error in=w115, "Defer Panel Updates"=w109) -> (reference out=w110:refnum<vi>, error out=w107:errorcluster)
        n216 = Close Reference(reference=w110, error in (no error)=w107) -> ()  [unwired: 1 out]
      }
      frame 2 {
        w549 = T1 1 items=["Exec Start", "Action completed", "pause to breath", "reserved 1", "reserved 2", "custom"] ("Call Reason")
      }
      frame 3, 4, Default {
      }
      frame 5 {
        n217 = while {
          shift-right: [w569] -> _
          shift-left: "Custom data" -> [w575]
          tunnel: "[\\s\\n]*;[\\s\\n]*" -> [w574]
          stop <- w568 stop-if-true
          n218 = Match Pattern(string=w575, regular expression=w574) -> (before substring=w573:string, after substring=w569:string)  [unwired: 1 in, 2 out]
          n219 = Empty String/Path?(string/path=w569) -> (empty?=w568:bool)
          n220 = Match Pattern(string=w573, regular expression="[\\s]*=[\\s]*") -> (before substring=w571:string, after substring=w570:string)  [unwired: 1 in, 2 out]
          n221 = case shown="\"LineMode\"" w571 {
            tunnel: w570 -> [_ w579]
            frame Default {
            }
            frame "LineMode" {
              n222 = To Upper Case(1:w579) -> (0:w578:string)
              n223 = Equal?(x=w578, y="TRUE") -> (x = y?=w576:bool)
              n224 = local write "Stepping mode"(w576) -> ()
            }
          }
        }
      }
    }
  }
  "Run Mode" <- w2
  "Breakpoints" <- w1
  "Stm Index out" <- w5
  "error out" <- "error in"
  "VC Handle out" <- "VC Handle"
  "dup CSE RefNum" <- "CSE RefNum"
